vi "Configure Module.vi"(8 "error in (no error)":errorcluster, 10 "IOV ref in":variant, 11 "Module Template in":refnum<class "SD Module.lvclass">) -> (0 "error out":errorcluster, 2 "IOV ref out":variant, 3 "Module Template out":refnum<class "SD Module.lvclass">)   [LabVIEW 2020, in "Modules.lvlib" / "SD Module.lvclass"]
uses:
  SD Module.lvclass
  <resource>/objmgr/cRIO.rc
  RSI Module/RSI Module.lvclass
  C:/Users/nitest/Desktop/Git 2020/niveristand-scan-engine-module-libraries/Source/RSI Module/RSI Module.lvclass
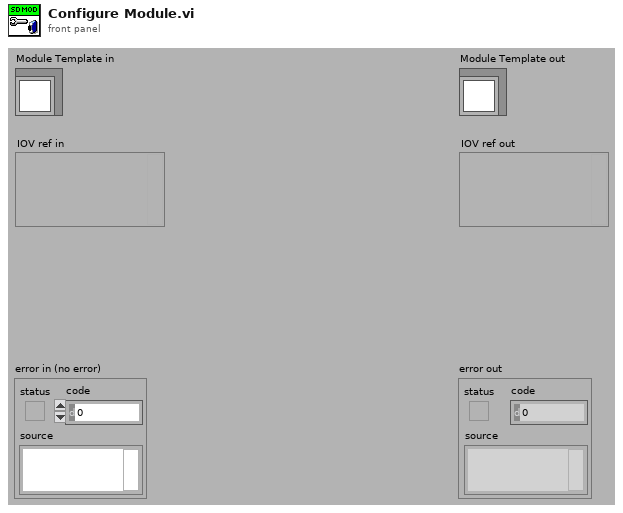
[diagram p1: front panel]
types:
  T1 = typedef "Modules.lvlib/SD Module.lvclass/Counter Channel.ctl" = cluster{"Measurement Mode":u32, "Count Edges":T2, "Period Measurement":T3, "Pulse Width Measurement":T4, "Frequency Measurement":T5}
  T2 = typedef "Modules.lvlib/SD Module.lvclass/Count Edges.ctl" = cluster{"Counter Event":u32, "Counter Source":u32, "Counter Direction":u32, "Terminal Count":u32, "Output Mode":u32, "Gate Mode":u32}
  T3 = typedef "Modules.lvlib/SD Module.lvclass/Period Measurement.ctl" = cluster{"Measurement Edge":u32}
  T4 = typedef "Modules.lvlib/SD Module.lvclass/Pulse Width Measurement.ctl" = cluster{"Measurement Type":u32}
  T5 = typedef "Modules.lvlib/SD Module.lvclass/Frequency Measurement.ctl" = cluster{"Measurement Edge":u32, "Measurement Timebase":u32}
  T6 = typedef "Modules.lvlib/SD Module.lvclass/CDO Channel.ctl" = cluster{"Counter driven enabled":bool}
  T7 = typedef "Modules.lvlib/SD Module.lvclass/PWM Channel.ctl" = cluster{"PWM frequency":u32}
  T8 = typedef "Modules.lvlib/SD Module.lvclass/Quadrature Channel.ctl" = cluster{"Timebase":u32, "Index Mode":u32}
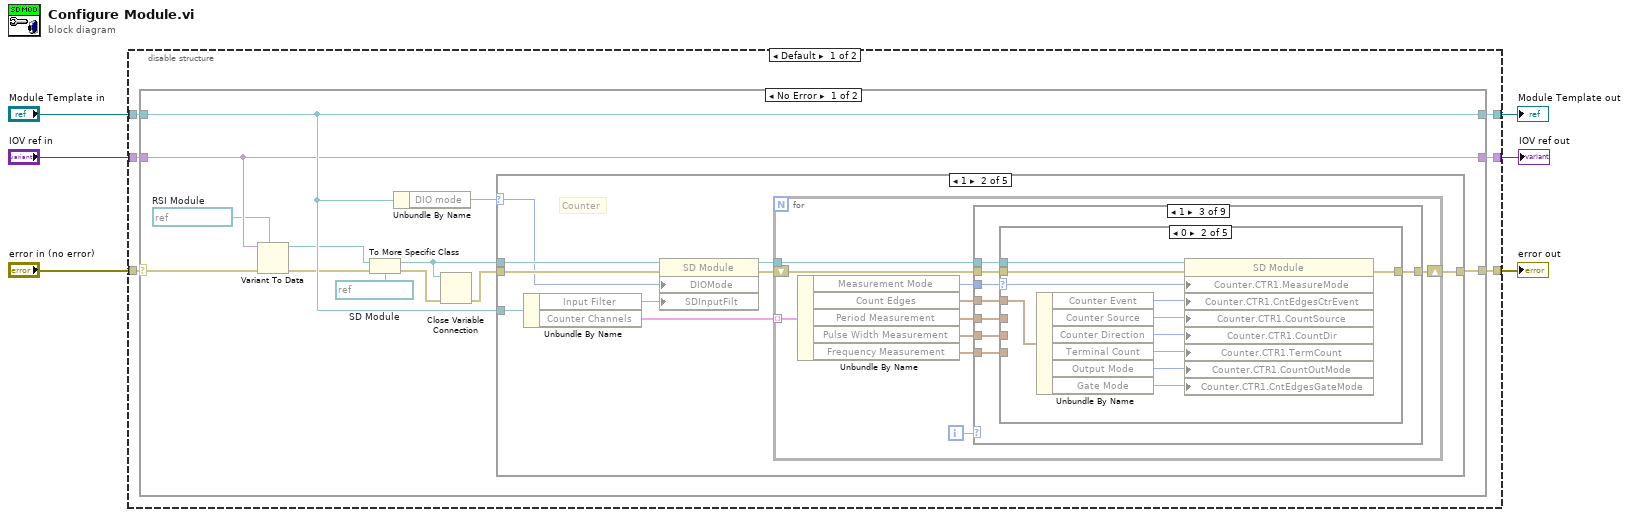
[diagram p0: block diagram]
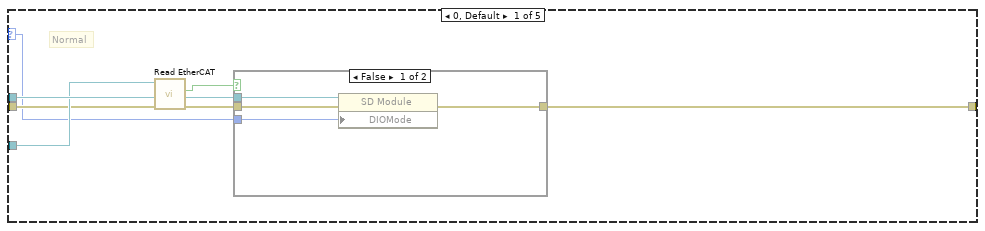
[diagram p2: hidden frame]
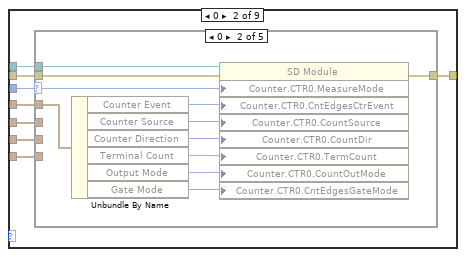
[diagram p5: hidden frame]
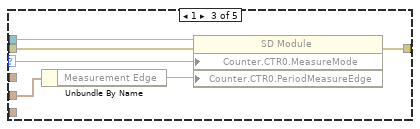
[diagram p7: hidden frame]
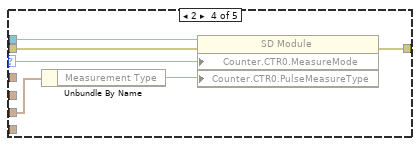
[diagram p8: hidden frame]
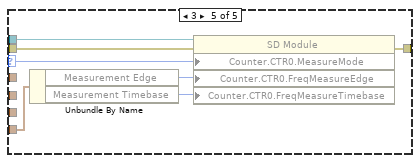
[diagram p9: hidden frame]
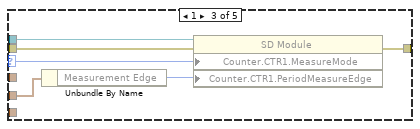
[diagram p11: hidden frame]
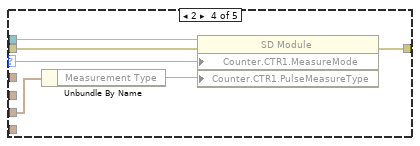
[diagram p12: hidden frame]
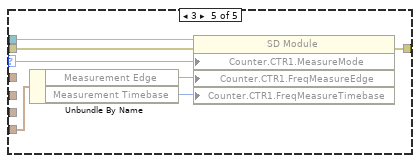
[diagram p13: hidden frame]
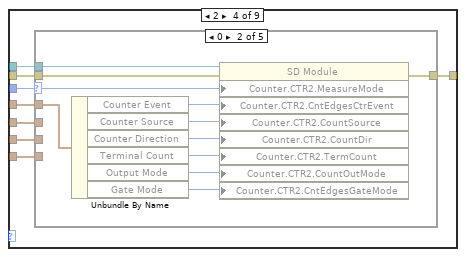
[diagram p14: hidden frame]
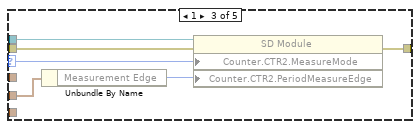
[diagram p16: hidden frame]
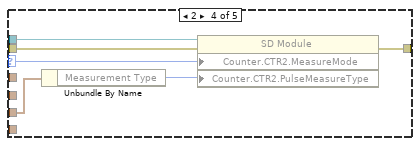
[diagram p17: hidden frame]
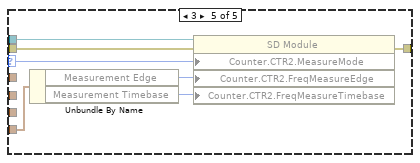
[diagram p18: hidden frame]
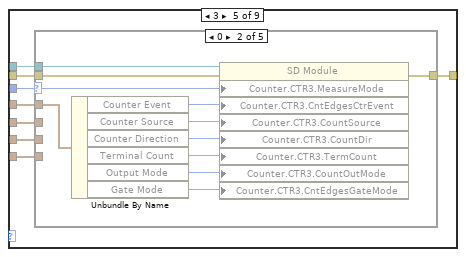
[diagram p19: hidden frame]
diagram:
  n1 = disable-structure shown="Default" {
    disable-tunnel: "error in (no error)" -> [w12 w494]
    disable-tunnel: [w11 w494] -> w5
    disable-tunnel: "Module Template in" -> [w10 w496]
    disable-tunnel: [w9 w496] -> w3
    disable-tunnel: "IOV ref in" -> [w8 w495]
    disable-tunnel: [w7 w495] -> w1
    frame condition #0 {
      n2 = case shown="No Error" w12 {
        selector: w12 -> [w16 w493]
        tunnel: [w18 w493] -> w11
        tunnel: [w19 w492] -> w9
        tunnel: w10 -> [w19 w492]
        tunnel: w8 -> [w17 w491]
        tunnel: [w17 w491] -> w7
        frame No Error {
          w13 = refnum<k21> refnum  # RSI Module
          w24 = refnum<k21> refnum  # SD Module
          n3 = Variant To Data(error in=w16, type=w13, Variant=w17) -> (data=w14:refnum<k21>, error out=w15:errorcluster)
          n4 = To More Specific Class(target class=w24, reference=w14, error in=w15) -> (specific class reference=w21:refnum<k21>, error out=w23:errorcluster)
          n5 = Unbundle By Name(w19) -> ("DIO mode"=w22:u32)
          n6 = Close Variable Connection(8:w23, 11:w21) -> (0:w20:errorcluster)
          n7 = case shown="1" w22 {
            selector: w22 -> [w25 w43 w375 w422 w470]
            tunnel: w21 -> [w31 w45 w377 w424 w472]
            tunnel: w20 -> [w27 w44 w376 w423 w471]
            tunnel: w19 -> [w29 w42 w374 w421 w469]
            tunnel: [w30 w37 w369 w417 w464] -> w18
            frame 0, Default {
              # "Normal"
              n8 = call "Read EtherCAT.vi"("error in (no error)"=w27, "RSI Module in"=w29) -> ("error out"=w26:errorcluster, "EtherCAT?"=w28:bool)  [unwired: 7 in, 1 out]
              n9 = case shown="False" w28 {
                tunnel: w31 -> [w35 _]
                tunnel: w26 -> [w34 w36]
                tunnel: [w33 w36] -> w30
                tunnel: w25 -> [w32 _]
                frame False {
                  n10 = property class="SD Module"(reference=w35, error in=w34, "DIOMode"=w32) -> (error out=w33:errorcluster)  [unwired: 1 out]
                }
                frame True {
                  # "Specialty Digital is not supported over\nEtherCAT, and explicitly configuring modules\nto use normal DIO mode will fail as a result."
                }
              }
            }
            frame 1 {
              # "Counter"
              n11 = Unbundle By Name(w42) -> ("Input Filter"=w41:u32, "Counter Channels"=w40:T1[])
              n12 = property class="SD Module"(reference=w45, error in=w44, "DIOMode"=w43, "SDInputFilt"=w41) -> (reference out=w39:refnum<k21>, error out=w38:errorcluster)
              n13 = for {
                tunnel: w40 -> [w51] mode=indexing
                tunnel: w39 -> [w54]
                shift-right: [w52] -> w37
                shift-left: w38 -> [w53]
                i -> [w55]
                n14 = Unbundle By Name(w51) -> ("Measurement Mode"=w50:u32, "Count Edges"=w49:T2, "Period Measurement"=w48:T3, "Pulse Width Measurement"=w47:T4, "Frequency Measurement"=w46:T5)
                n15 = case shown="1" w55 {
                  tunnel: w54 -> [_ w59 w98 w137 w176 w215 w254 w293 w332]
                  tunnel: w53 -> [w56 w58 w97 w136 w175 w214 w253 w292 w331]
                  tunnel: [w56 w57 w96 w135 w174 w213 w252 w291 w330] -> w52
                  tunnel: w50 -> [_ w64 w103 w142 w181 w220 w259 w298 w337]
                  tunnel: w49 -> [_ w63 w102 w141 w180 w219 w258 w297 w336]
                  tunnel: w48 -> [_ w62 w101 w140 w179 w218 w257 w296 w335]
                  tunnel: w47 -> [_ w61 w100 w139 w178 w217 w256 w295 w334]
                  tunnel: w46 -> [_ w60 w99 w138 w177 w216 w255 w294 w333]
                  frame Default {
                  }
                  frame 0 {
                    n16 = case shown="0" w64 {
                      selector: w64 -> [_ w73 w80 w86 w93]
                      tunnel: w63 -> [_ w76 _ _ _]
                      tunnel: w62 -> [_ _ w77 _ _]
                      tunnel: w61 -> [_ _ _ w83 _]
                      tunnel: w60 -> [_ _ _ _ w90]
                      tunnel: w59 -> [_ w75 w82 w88 w95]
                      tunnel: w58 -> [w65 w74 w81 w87 w94]
                      tunnel: [w65 w66 w78 w84 w91] -> w57
                      frame Default {
                      }
                      frame 0 {
                        n17 = Unbundle By Name(w76) -> ("Counter Event"=w72:u32, "Counter Source"=w71:u32, "Counter Direction"=w70:u32, "Terminal Count"=w69:u32, "Output Mode"=w68:u32, "Gate Mode"=w67:u32)
                        n18 = property class="SD Module"(reference=w75, error in=w74, "Counter.CTR0.MeasureMode"=w73, "Counter.CTR0.CntEdgesCtrEvent"=w72, "Counter.CTR0.CountSource"=w71, "Counter.CTR0.CountDir"=w70, "Counter.CTR0.TermCount"=w69, "Counter.CTR0.CountOutMode"=w68, "Counter.CTR0.CntEdgesGateMode"=w67) -> (error out=w66:errorcluster)  [unwired: 1 out]
                      }
                      frame 1 {
                        n19 = Unbundle By Name(w77) -> ("Measurement Edge"=w79:u32)
                        n20 = property class="SD Module"(reference=w82, error in=w81, "Counter.CTR0.MeasureMode"=w80, "Counter.CTR0.PeriodMeasureEdge"=w79) -> (error out=w78:errorcluster)  [unwired: 1 out]
                      }
                      frame 2 {
                        n21 = Unbundle By Name(w83) -> ("Measurement Type"=w85:u32)
                        n22 = property class="SD Module"(reference=w88, error in=w87, "Counter.CTR0.MeasureMode"=w86, "Counter.CTR0.PulseMeasureType"=w85) -> (error out=w84:errorcluster)  [unwired: 1 out]
                      }
                      frame 3 {
                        n23 = Unbundle By Name(w90) -> ("Measurement Edge"=w92:u32, "Measurement Timebase"=w89:u32)
                        n24 = property class="SD Module"(reference=w95, error in=w94, "Counter.CTR0.MeasureMode"=w93, "Counter.CTR0.FreqMeasureEdge"=w92, "Counter.CTR0.FreqMeasureTimebase"=w89) -> (error out=w91:errorcluster)  [unwired: 1 out]
                      }
                    }
                  }
                  frame 1 {
                    n25 = case shown="0" w103 {
                      selector: w103 -> [_ w112 w119 w125 w132]
                      tunnel: w102 -> [_ w115 _ _ _]
                      tunnel: w101 -> [_ _ w116 _ _]
                      tunnel: w100 -> [_ _ _ w122 _]
                      tunnel: w99 -> [_ _ _ _ w129]
                      tunnel: w98 -> [_ w114 w121 w127 w134]
                      tunnel: w97 -> [w104 w113 w120 w126 w133]
                      tunnel: [w104 w105 w117 w123 w130] -> w96
                      frame Default {
                      }
                      frame 0 {
                        n26 = Unbundle By Name(w115) -> ("Counter Event"=w111:u32, "Counter Source"=w110:u32, "Counter Direction"=w109:u32, "Terminal Count"=w108:u32, "Output Mode"=w107:u32, "Gate Mode"=w106:u32)
                        n27 = property class="SD Module"(reference=w114, error in=w113, "Counter.CTR1.MeasureMode"=w112, "Counter.CTR1.CntEdgesCtrEvent"=w111, "Counter.CTR1.CountSource"=w110, "Counter.CTR1.CountDir"=w109, "Counter.CTR1.TermCount"=w108, "Counter.CTR1.CountOutMode"=w107, "Counter.CTR1.CntEdgesGateMode"=w106) -> (error out=w105:errorcluster)  [unwired: 1 out]
                      }
                      frame 1 {
                        n28 = Unbundle By Name(w116) -> ("Measurement Edge"=w118:u32)
                        n29 = property class="SD Module"(reference=w121, error in=w120, "Counter.CTR1.MeasureMode"=w119, "Counter.CTR1.PeriodMeasureEdge"=w118) -> (error out=w117:errorcluster)  [unwired: 1 out]
                      }
                      frame 2 {
                        n30 = Unbundle By Name(w122) -> ("Measurement Type"=w124:u32)
                        n31 = property class="SD Module"(reference=w127, error in=w126, "Counter.CTR1.MeasureMode"=w125, "Counter.CTR1.PulseMeasureType"=w124) -> (error out=w123:errorcluster)  [unwired: 1 out]
                      }
                      frame 3 {
                        n32 = Unbundle By Name(w129) -> ("Measurement Edge"=w131:u32, "Measurement Timebase"=w128:u32)
                        n33 = property class="SD Module"(reference=w134, error in=w133, "Counter.CTR1.MeasureMode"=w132, "Counter.CTR1.FreqMeasureEdge"=w131, "Counter.CTR1.FreqMeasureTimebase"=w128) -> (error out=w130:errorcluster)  [unwired: 1 out]
                      }
                    }
                  }
                  frame 2 {
                    n34 = case shown="0" w142 {
                      selector: w142 -> [_ w151 w158 w164 w171]
                      tunnel: w141 -> [_ w154 _ _ _]
                      tunnel: w140 -> [_ _ w155 _ _]
                      tunnel: w139 -> [_ _ _ w161 _]
                      tunnel: w138 -> [_ _ _ _ w168]
                      tunnel: w137 -> [_ w153 w160 w166 w173]
                      tunnel: w136 -> [w143 w152 w159 w165 w172]
                      tunnel: [w143 w144 w156 w162 w169] -> w135
                      frame Default {
                      }
                      frame 0 {
                        n35 = Unbundle By Name(w154) -> ("Counter Event"=w150:u32, "Counter Source"=w149:u32, "Counter Direction"=w148:u32, "Terminal Count"=w147:u32, "Output Mode"=w146:u32, "Gate Mode"=w145:u32)
                        n36 = property class="SD Module"(reference=w153, error in=w152, "Counter.CTR2.MeasureMode"=w151, "Counter.CTR2.CntEdgesCtrEvent"=w150, "Counter.CTR2.CountSource"=w149, "Counter.CTR2.CountDir"=w148, "Counter.CTR2.TermCount"=w147, "Counter.CTR2.CountOutMode"=w146, "Counter.CTR2.CntEdgesGateMode"=w145) -> (error out=w144:errorcluster)  [unwired: 1 out]
                      }
                      frame 1 {
                        n37 = Unbundle By Name(w155) -> ("Measurement Edge"=w157:u32)
                        n38 = property class="SD Module"(reference=w160, error in=w159, "Counter.CTR2.MeasureMode"=w158, "Counter.CTR2.PeriodMeasureEdge"=w157) -> (error out=w156:errorcluster)  [unwired: 1 out]
                      }
                      frame 2 {
                        n39 = Unbundle By Name(w161) -> ("Measurement Type"=w163:u32)
                        n40 = property class="SD Module"(reference=w166, error in=w165, "Counter.CTR2.MeasureMode"=w164, "Counter.CTR2.PulseMeasureType"=w163) -> (error out=w162:errorcluster)  [unwired: 1 out]
                      }
                      frame 3 {
                        n41 = Unbundle By Name(w168) -> ("Measurement Edge"=w170:u32, "Measurement Timebase"=w167:u32)
                        n42 = property class="SD Module"(reference=w173, error in=w172, "Counter.CTR2.MeasureMode"=w171, "Counter.CTR2.FreqMeasureEdge"=w170, "Counter.CTR2.FreqMeasureTimebase"=w167) -> (error out=w169:errorcluster)  [unwired: 1 out]
                      }
                    }
                  }
                  frame 3 {
                    n43 = case shown="0" w181 {
                      selector: w181 -> [_ w190 w197 w203 w210]
                      tunnel: w180 -> [_ w193 _ _ _]
                      tunnel: w179 -> [_ _ w194 _ _]
                      tunnel: w178 -> [_ _ _ w200 _]
                      tunnel: w177 -> [_ _ _ _ w207]
                      tunnel: w176 -> [_ w192 w199 w205 w212]
                      tunnel: w175 -> [w182 w191 w198 w204 w211]
                      tunnel: [w182 w183 w195 w201 w208] -> w174
                      frame Default {
                      }
                      frame 0 {
                        n44 = Unbundle By Name(w193) -> ("Counter Event"=w189:u32, "Counter Source"=w188:u32, "Counter Direction"=w187:u32, "Terminal Count"=w186:u32, "Output Mode"=w185:u32, "Gate Mode"=w184:u32)
                        n45 = property class="SD Module"(reference=w192, error in=w191, "Counter.CTR3.MeasureMode"=w190, "Counter.CTR3.CntEdgesCtrEvent"=w189, "Counter.CTR3.CountSource"=w188, "Counter.CTR3.CountDir"=w187, "Counter.CTR3.TermCount"=w186, "Counter.CTR3.CountOutMode"=w185, "Counter.CTR3.CntEdgesGateMode"=w184) -> (error out=w183:errorcluster)  [unwired: 1 out]
                      }
                      frame 1 {
                        n46 = Unbundle By Name(w194) -> ("Measurement Edge"=w196:u32)
                        n47 = property class="SD Module"(reference=w199, error in=w198, "Counter.CTR3.MeasureMode"=w197, "Counter.CTR3.PeriodMeasureEdge"=w196) -> (error out=w195:errorcluster)  [unwired: 1 out]
                      }
                      frame 2 {
                        n48 = Unbundle By Name(w200) -> ("Measurement Type"=w202:u32)
                        n49 = property class="SD Module"(reference=w205, error in=w204, "Counter.CTR3.MeasureMode"=w203, "Counter.CTR3.PulseMeasureType"=w202) -> (error out=w201:errorcluster)  [unwired: 1 out]
                      }
                      frame 3 {
                        n50 = Unbundle By Name(w207) -> ("Measurement Edge"=w209:u32, "Measurement Timebase"=w206:u32)
                        n51 = property class="SD Module"(reference=w212, error in=w211, "Counter.CTR3.MeasureMode"=w210, "Counter.CTR3.FreqMeasureEdge"=w209, "Counter.CTR3.FreqMeasureTimebase"=w206) -> (error out=w208:errorcluster)  [unwired: 1 out]
                      }
                    }
                  }
                  frame 4 {
                    n52 = case shown="0" w220 {
                      selector: w220 -> [_ w229 w236 w242 w249]
                      tunnel: w219 -> [_ w232 _ _ _]
                      tunnel: w218 -> [_ _ w233 _ _]
                      tunnel: w217 -> [_ _ _ w239 _]
                      tunnel: w216 -> [_ _ _ _ w246]
                      tunnel: w215 -> [_ w231 w238 w244 w251]
                      tunnel: w214 -> [w221 w230 w237 w243 w250]
                      tunnel: [w221 w222 w234 w240 w247] -> w213
                      frame Default {
                      }
                      frame 0 {
                        n53 = Unbundle By Name(w232) -> ("Counter Event"=w228:u32, "Counter Source"=w227:u32, "Counter Direction"=w226:u32, "Terminal Count"=w225:u32, "Output Mode"=w224:u32, "Gate Mode"=w223:u32)
                        n54 = property class="SD Module"(reference=w231, error in=w230, "Counter.CTR4.MeasureMode"=w229, "Counter.CTR4.CntEdgesCtrEvent"=w228, "Counter.CTR4.CountSource"=w227, "Counter.CTR4.CountDir"=w226, "Counter.CTR4.TermCount"=w225, "Counter.CTR4.CountOutMode"=w224, "Counter.CTR4.CntEdgesGateMode"=w223) -> (error out=w222:errorcluster)  [unwired: 1 out]
                      }
                      frame 1 {
                        n55 = Unbundle By Name(w233) -> ("Measurement Edge"=w235:u32)
                        n56 = property class="SD Module"(reference=w238, error in=w237, "Counter.CTR4.MeasureMode"=w236, "Counter.CTR4.PeriodMeasureEdge"=w235) -> (error out=w234:errorcluster)  [unwired: 1 out]
                      }
                      frame 2 {
                        n57 = Unbundle By Name(w239) -> ("Measurement Type"=w241:u32)
                        n58 = property class="SD Module"(reference=w244, error in=w243, "Counter.CTR4.MeasureMode"=w242, "Counter.CTR4.PulseMeasureType"=w241) -> (error out=w240:errorcluster)  [unwired: 1 out]
                      }
                      frame 3 {
                        n59 = Unbundle By Name(w246) -> ("Measurement Edge"=w248:u32, "Measurement Timebase"=w245:u32)
                        n60 = property class="SD Module"(reference=w251, error in=w250, "Counter.CTR4.MeasureMode"=w249, "Counter.CTR4.FreqMeasureEdge"=w248, "Counter.CTR4.FreqMeasureTimebase"=w245) -> (error out=w247:errorcluster)  [unwired: 1 out]
                      }
                    }
                  }
                  frame 5 {
                    n61 = case shown="0" w259 {
                      selector: w259 -> [_ w268 w275 w281 w288]
                      tunnel: w258 -> [_ w271 _ _ _]
                      tunnel: w257 -> [_ _ w272 _ _]
                      tunnel: w256 -> [_ _ _ w278 _]
                      tunnel: w255 -> [_ _ _ _ w285]
                      tunnel: w254 -> [_ w270 w277 w283 w290]
                      tunnel: w253 -> [w260 w269 w276 w282 w289]
                      tunnel: [w260 w261 w273 w279 w286] -> w252
                      frame Default {
                      }
                      frame 0 {
                        n62 = Unbundle By Name(w271) -> ("Counter Event"=w267:u32, "Counter Source"=w266:u32, "Counter Direction"=w265:u32, "Terminal Count"=w264:u32, "Output Mode"=w263:u32, "Gate Mode"=w262:u32)
                        n63 = property class="SD Module"(reference=w270, error in=w269, "Counter.CTR5.MeasureMode"=w268, "Counter.CTR5.CntEdgesCtrEvent"=w267, "Counter.CTR5.CountSource"=w266, "Counter.CTR5.CountDir"=w265, "Counter.CTR5.TermCount"=w264, "Counter.CTR5.CountOutMode"=w263, "Counter.CTR5.CntEdgesGateMode"=w262) -> (error out=w261:errorcluster)  [unwired: 1 out]
                      }
                      frame 1 {
                        n64 = Unbundle By Name(w272) -> ("Measurement Edge"=w274:u32)
                        n65 = property class="SD Module"(reference=w277, error in=w276, "Counter.CTR5.MeasureMode"=w275, "Counter.CTR5.PeriodMeasureEdge"=w274) -> (error out=w273:errorcluster)  [unwired: 1 out]
                      }
                      frame 2 {
                        n66 = Unbundle By Name(w278) -> ("Measurement Type"=w280:u32)
                        n67 = property class="SD Module"(reference=w283, error in=w282, "Counter.CTR5.MeasureMode"=w281, "Counter.CTR5.PulseMeasureType"=w280) -> (error out=w279:errorcluster)  [unwired: 1 out]
                      }
                      frame 3 {
                        n68 = Unbundle By Name(w285) -> ("Measurement Edge"=w287:u32, "Measurement Timebase"=w284:u32)
                        n69 = property class="SD Module"(reference=w290, error in=w289, "Counter.CTR5.MeasureMode"=w288, "Counter.CTR5.FreqMeasureEdge"=w287, "Counter.CTR5.FreqMeasureTimebase"=w284) -> (error out=w286:errorcluster)  [unwired: 1 out]
                      }
                    }
                  }
                  frame 6 {
                    n70 = case shown="0" w298 {
                      selector: w298 -> [_ w307 w314 w320 w327]
                      tunnel: w297 -> [_ w310 _ _ _]
                      tunnel: w296 -> [_ _ w311 _ _]
                      tunnel: w295 -> [_ _ _ w317 _]
                      tunnel: w294 -> [_ _ _ _ w324]
                      tunnel: w293 -> [_ w309 w316 w322 w329]
                      tunnel: w292 -> [w299 w308 w315 w321 w328]
                      tunnel: [w299 w300 w312 w318 w325] -> w291
                      frame Default {
                      }
                      frame 0 {
                        n71 = Unbundle By Name(w310) -> ("Counter Event"=w306:u32, "Counter Source"=w305:u32, "Counter Direction"=w304:u32, "Terminal Count"=w303:u32, "Output Mode"=w302:u32, "Gate Mode"=w301:u32)
                        n72 = property class="SD Module"(reference=w309, error in=w308, "Counter.CTR6.MeasureMode"=w307, "Counter.CTR6.CntEdgesCtrEvent"=w306, "Counter.CTR6.CountSource"=w305, "Counter.CTR6.CountDir"=w304, "Counter.CTR6.TermCount"=w303, "Counter.CTR6.CountOutMode"=w302, "Counter.CTR6.CntEdgesGateMode"=w301) -> (error out=w300:errorcluster)  [unwired: 1 out]
                      }
                      frame 1 {
                        n73 = Unbundle By Name(w311) -> ("Measurement Edge"=w313:u32)
                        n74 = property class="SD Module"(reference=w316, error in=w315, "Counter.CTR6.MeasureMode"=w314, "Counter.CTR6.PeriodMeasureEdge"=w313) -> (error out=w312:errorcluster)  [unwired: 1 out]
                      }
                      frame 2 {
                        n75 = Unbundle By Name(w317) -> ("Measurement Type"=w319:u32)
                        n76 = property class="SD Module"(reference=w322, error in=w321, "Counter.CTR6.MeasureMode"=w320, "Counter.CTR6.PulseMeasureType"=w319) -> (error out=w318:errorcluster)  [unwired: 1 out]
                      }
                      frame 3 {
                        n77 = Unbundle By Name(w324) -> ("Measurement Edge"=w326:u32, "Measurement Timebase"=w323:u32)
                        n78 = property class="SD Module"(reference=w329, error in=w328, "Counter.CTR6.MeasureMode"=w327, "Counter.CTR6.FreqMeasureEdge"=w326, "Counter.CTR6.FreqMeasureTimebase"=w323) -> (error out=w325:errorcluster)  [unwired: 1 out]
                      }
                    }
                  }
                  frame 7 {
                    n79 = case shown="0" w337 {
                      selector: w337 -> [_ w346 w353 w359 w366]
                      tunnel: w336 -> [_ w349 _ _ _]
                      tunnel: w335 -> [_ _ w350 _ _]
                      tunnel: w334 -> [_ _ _ w356 _]
                      tunnel: w333 -> [_ _ _ _ w363]
                      tunnel: w332 -> [_ w348 w355 w361 w368]
                      tunnel: w331 -> [w338 w347 w354 w360 w367]
                      tunnel: [w338 w339 w351 w357 w364] -> w330
                      frame Default {
                      }
                      frame 0 {
                        n80 = Unbundle By Name(w349) -> ("Counter Event"=w345:u32, "Counter Source"=w344:u32, "Counter Direction"=w343:u32, "Terminal Count"=w342:u32, "Output Mode"=w341:u32, "Gate Mode"=w340:u32)
                        n81 = property class="SD Module"(reference=w348, error in=w347, "Counter.CTR7.MeasureMode"=w346, "Counter.CTR7.CntEdgesCtrEvent"=w345, "Counter.CTR7.CountSource"=w344, "Counter.CTR7.CountDir"=w343, "Counter.CTR7.TermCount"=w342, "Counter.CTR7.CountOutMode"=w341, "Counter.CTR7.CntEdgesGateMode"=w340) -> (error out=w339:errorcluster)  [unwired: 1 out]
                      }
                      frame 1 {
                        n82 = Unbundle By Name(w350) -> ("Measurement Edge"=w352:u32)
                        n83 = property class="SD Module"(reference=w355, error in=w354, "Counter.CTR7.MeasureMode"=w353, "Counter.CTR7.PeriodMeasureEdge"=w352) -> (error out=w351:errorcluster)  [unwired: 1 out]
                      }
                      frame 2 {
                        n84 = Unbundle By Name(w356) -> ("Measurement Type"=w358:u32)
                        n85 = property class="SD Module"(reference=w361, error in=w360, "Counter.CTR7.MeasureMode"=w359, "Counter.CTR7.PulseMeasureType"=w358) -> (error out=w357:errorcluster)  [unwired: 1 out]
                      }
                      frame 3 {
                        n86 = Unbundle By Name(w363) -> ("Measurement Edge"=w365:u32, "Measurement Timebase"=w362:u32)
                        n87 = property class="SD Module"(reference=w368, error in=w367, "Counter.CTR7.MeasureMode"=w366, "Counter.CTR7.FreqMeasureEdge"=w365, "Counter.CTR7.FreqMeasureTimebase"=w362) -> (error out=w364:errorcluster)  [unwired: 1 out]
                      }
                    }
                  }
                }
              }
            }
            frame 2 {
              # "Counter-Driven Output"
              n88 = Unbundle By Name(w374) -> ("Drive From Slot"=w371:u32, "CDO Channels"=w370:T6[])
              n89 = property class="SD Module"(reference=w377, error in=w376, "DIOMode"=w375, "CDO.CountSlvMastSlot"=w371) -> (reference out=w373:refnum<k21>, error out=w372:errorcluster)
              n90 = for {
                tunnel: w373 -> [w382]
                shift-right: [w380] -> w369
                shift-left: w372 -> [w381]
                tunnel: w370 -> [w378] mode=indexing
                i -> [w383]
                n91 = Unbundle By Name(w378) -> ("Counter driven enabled"=w379:bool)
                n92 = case shown="0" w383 {
                  tunnel: w382 -> [_ w388 w392 w396 w400 w404 w408 w412 w416]
                  tunnel: w381 -> [w384 w387 w391 w395 w399 w403 w407 w411 w415]
                  tunnel: [w384 w386 w390 w394 w398 w402 w406 w410 w414] -> w380
                  tunnel: w379 -> [_ w385 w389 w393 w397 w401 w405 w409 w413]
                  frame Default {
                  }
                  frame 0 {
                    n93 = property class="SD Module"(reference=w388, error in=w387, "CDO.CTR0.CtrDrivenEnabled"=w385) -> (error out=w386:errorcluster)  [unwired: 1 out]
                  }
                  frame 1 {
                    n94 = property class="SD Module"(reference=w392, error in=w391, "CDO.CTR1.CtrDrivenEnabled"=w389) -> (error out=w390:errorcluster)  [unwired: 1 out]
                  }
                  frame 2 {
                    n95 = property class="SD Module"(reference=w396, error in=w395, "CDO.CTR2.CtrDrivenEnabled"=w393) -> (error out=w394:errorcluster)  [unwired: 1 out]
                  }
                  frame 3 {
                    n96 = property class="SD Module"(reference=w400, error in=w399, "CDO.CTR3.CtrDrivenEnabled"=w397) -> (error out=w398:errorcluster)  [unwired: 1 out]
                  }
                  frame 4 {
                    n97 = property class="SD Module"(reference=w404, error in=w403, "CDO.CTR4.CtrDrivenEnabled"=w401) -> (error out=w402:errorcluster)  [unwired: 1 out]
                  }
                  frame 5 {
                    n98 = property class="SD Module"(reference=w408, error in=w407, "CDO.CTR5.CtrDrivenEnabled"=w405) -> (error out=w406:errorcluster)  [unwired: 1 out]
                  }
                  frame 6 {
                    n99 = property class="SD Module"(reference=w412, error in=w411, "CDO.CTR6.CtrDrivenEnabled"=w409) -> (error out=w410:errorcluster)  [unwired: 1 out]
                  }
                  frame 7 {
                    n100 = property class="SD Module"(reference=w416, error in=w415, "CDO.CTR7.CtrDrivenEnabled"=w413) -> (error out=w414:errorcluster)  [unwired: 1 out]
                  }
                }
              }
            }
            frame 3 {
              # "Pulse-Width Modulation"
              n101 = Unbundle By Name(w421) -> ("PWM Channels"=w418:T7[])
              n102 = property class="SD Module"(reference=w424, error in=w423, "DIOMode"=w422) -> (reference out=w420:refnum<k21>, error out=w419:errorcluster)
              n103 = for {
                tunnel: w420 -> [w429]
                shift-right: [w427] -> w417
                shift-left: w419 -> [w428]
                tunnel: w418 -> [w425] mode=indexing
                i -> [w430]
                n104 = Unbundle By Name(w425) -> ("PWM frequency"=w426:u32)
                n105 = case shown="0" w430 {
                  tunnel: w429 -> [_ w435 w439 w443 w447 w451 w455 w459 w463]
                  tunnel: w428 -> [w431 w434 w438 w442 w446 w450 w454 w458 w462]
                  tunnel: [w431 w433 w437 w441 w445 w449 w453 w457 w461] -> w427
                  tunnel: w426 -> [_ w432 w436 w440 w444 w448 w452 w456 w460]
                  frame Default {
                  }
                  frame 0 {
                    n106 = property class="SD Module"(reference=w435, error in=w434, "PWM.PWM0.PWMFrequency"=w432) -> (error out=w433:errorcluster)  [unwired: 1 out]
                  }
                  frame 1 {
                    n107 = property class="SD Module"(reference=w439, error in=w438, "PWM.PWM1.PWMFrequency"=w436) -> (error out=w437:errorcluster)  [unwired: 1 out]
                  }
                  frame 2 {
                    n108 = property class="SD Module"(reference=w443, error in=w442, "PWM.PWM2.PWMFrequency"=w440) -> (error out=w441:errorcluster)  [unwired: 1 out]
                  }
                  frame 3 {
                    n109 = property class="SD Module"(reference=w447, error in=w446, "PWM.PWM3.PWMFrequency"=w444) -> (error out=w445:errorcluster)  [unwired: 1 out]
                  }
                  frame 4 {
                    n110 = property class="SD Module"(reference=w451, error in=w450, "PWM.PWM4.PWMFrequency"=w448) -> (error out=w449:errorcluster)  [unwired: 1 out]
                  }
                  frame 5 {
                    n111 = property class="SD Module"(reference=w455, error in=w454, "PWM.PWM5.PWMFrequency"=w452) -> (error out=w453:errorcluster)  [unwired: 1 out]
                  }
                  frame 6 {
                    n112 = property class="SD Module"(reference=w459, error in=w458, "PWM.PWM6.PWMFrequency"=w456) -> (error out=w457:errorcluster)  [unwired: 1 out]
                  }
                  frame 7 {
                    n113 = property class="SD Module"(reference=w463, error in=w462, "PWM.PWM7.PWMFrequency"=w460) -> (error out=w461:errorcluster)  [unwired: 1 out]
                  }
                }
              }
            }
            frame 4 {
              # "Quadrature"
              n114 = Unbundle By Name(w469) -> ("Input Filter"=w468:u32, "Quadrature Channels"=w467:T8[])
              n115 = property class="SD Module"(reference=w472, error in=w471, "DIOMode"=w470, "SDInputFilt"=w468) -> (reference out=w466:refnum<k21>, error out=w465:errorcluster)
              n116 = for {
                tunnel: w467 -> [w475] mode=indexing
                tunnel: w466 -> [w478]
                shift-right: [w476] -> w464
                shift-left: w465 -> [w477]
                i -> [w479]
                n117 = Unbundle By Name(w475) -> ("Timebase"=w474:u32, "Index Mode"=w473:u32)
                n118 = case shown="0" w479 {
                  tunnel: w478 -> [_ w485 w490]
                  tunnel: w477 -> [w480 w484 w489]
                  tunnel: [w480 w483 w488] -> w476
                  tunnel: w474 -> [_ w482 w487]
                  tunnel: w473 -> [_ w481 w486]
                  frame Default {
                  }
                  frame 0 {
                    n119 = property class="SD Module"(reference=w485, error in=w484, "Quad.Quadrature0.QuadTimebase"=w482, "Quad.Quadrature0.QuadIdxMode"=w481) -> (error out=w483:errorcluster)  [unwired: 1 out]
                  }
                  frame 1 {
                    n120 = property class="SD Module"(reference=w490, error in=w489, "Quad.Quadrature1.QuadTimebase"=w487, "Quad.Quadrature0.QuadIdxMode"=w486) -> (error out=w488:errorcluster)  [unwired: 1 out]
                  }
                }
              }
            }
          }
        }
        frame Error {
        }
      }
    }
    frame condition #1 (active) {
    }
  }
  "error out" <- w5
  "Module Template out" <- w3
  "IOV ref out" <- w1
